vi "TimeConstantFilter_Example.vi"() -> ()   [LabVIEW 2019]
uses:
  <vilib>/Rock Robotics/WPI/ThirdParty/JAS_Junk/TrajLib/Trajectory_Library.lvlib
  <vilib>/Rock Robotics/WPI/ThirdParty/JAS_Junk/TrajLib/LinearFilter_LP_BW1_Execute.vi
  <vilib>/Rock Robotics/WPI/ThirdParty/JAS_Junk/TrajLib/LinearFilter_LP_BW2_Execute.vi
  <vilib>/Rock Robotics/WPI/ThirdParty/JAS_Junk/TrajLib/LinearFilter_HP_BW1_Execute.vi
  <vilib>/Rock Robotics/WPI/ThirdParty/JAS_Junk/TrajLib/LinearFilter_HP_BW2_Execute.vi
panel:
  out "Wait Adjust":dbl format="%11.3f"
  in  "Auto / Manual":bool=TRUE
  in  "Enable\nNoise":bool=TRUE
  in  "Filter Enable":bool=TRUE
  in  "Use White Noise":bool=TRUE
  in  "Tab Control 2":T1(tab)
  out "LP BW 2":cluster{dbl, dbl, "Output_Value":dbl}(graph)
  out "Butter 1 Out":dbl format="%11.3f"
  out "Low Pass Butterworth 1 Dial":dbl(knob)=-2.895988890827539e-05 scale=-20.0..20.0
  out "Curoff Freq\nLP BW 1":dbl format="%11.3f"
  out "LP BW 2":cluster{dbl, dbl, "Output_Value":dbl}(graph)
  out "Butter 2 Out":dbl format="%11.3f"
  out "Low Pass Butterworth 2 Dial":dbl(knob)=-2.895988890827539e-05 scale=-20.0..20.0
  out "Cutoff  Freq\nLP BW 2":dbl format="%11.3f"
  out "Curoff Freq\nHP BW 1":dbl format="%11.3f"
  out "HP BW 1":cluster{dbl, dbl, "Output_Value":dbl}(graph)
  out "HP BW 1":dbl format="%11.3f"
  out "High Pass Butterworth 1":dbl(knob)=-2.895988890827539e-05 scale=-20.0..20.0
  out "HP  BW 2":cluster{dbl, dbl, "Output_Value":dbl}(graph)
  out "Alt Lag":dbl format="%11.3f"
  out "High Pass Butterworth 2":dbl(knob)=-2.895988890827539e-05 scale=-20.0..20.0
  out "Cutoff Freq\nHP BW 2":dbl format="%11.3f"
  out "Duration":dbl format="%11.3f"
  out "Late":dbl format="%11.3f"
  in  "Manual\nInput":dbl(slide) min=-12.0 max=12.0 scale=-12.0..12.0
  out "Raw Noise":dbl(knob)=-2.895988890827539e-05 scale=-20.0..20.0
  out "Raw Noise":dbl format="%11.3f"
  out "Actual Input":dbl(knob)=-2.895988890827539e-05 scale=-20.0..20.0
  out "Actual Input":dbl format="%11.3f"
  in  "Time Const (Sec)":dbl=0.08 min=0.0 step=0.001 format="%10.4f"
  out "Input":cluster{"Manual\nInput":dbl, dbl, "f":dbl}(graph)
  out "Meas Dial":dbl(knob)=-2.895988890827539e-05 scale=-20.0..20.0
  out "Measured Value":dbl format="%11.3f"
  # "Linear (Time Constant) Filter Example"
  # "Loop Information"
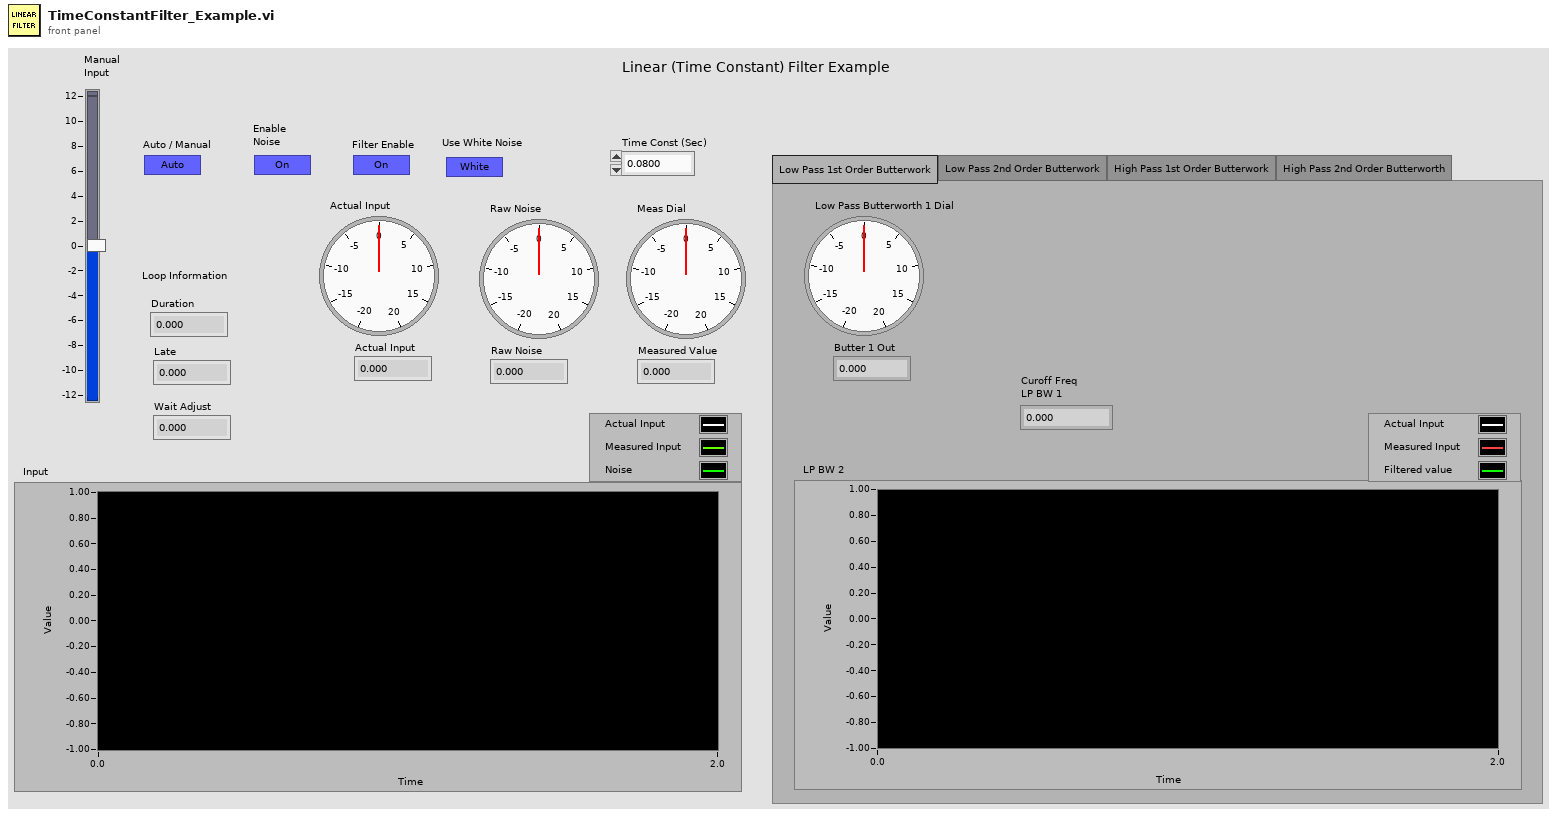
[diagram p1: front panel]
types:
  T1 = enum32{"Low Pass 1st Order Butterwork", "Low Pass 2nd Order Butterwork", "High Pass 1st Order Butterwork", "High Pass 2nd Order Butterworth"}
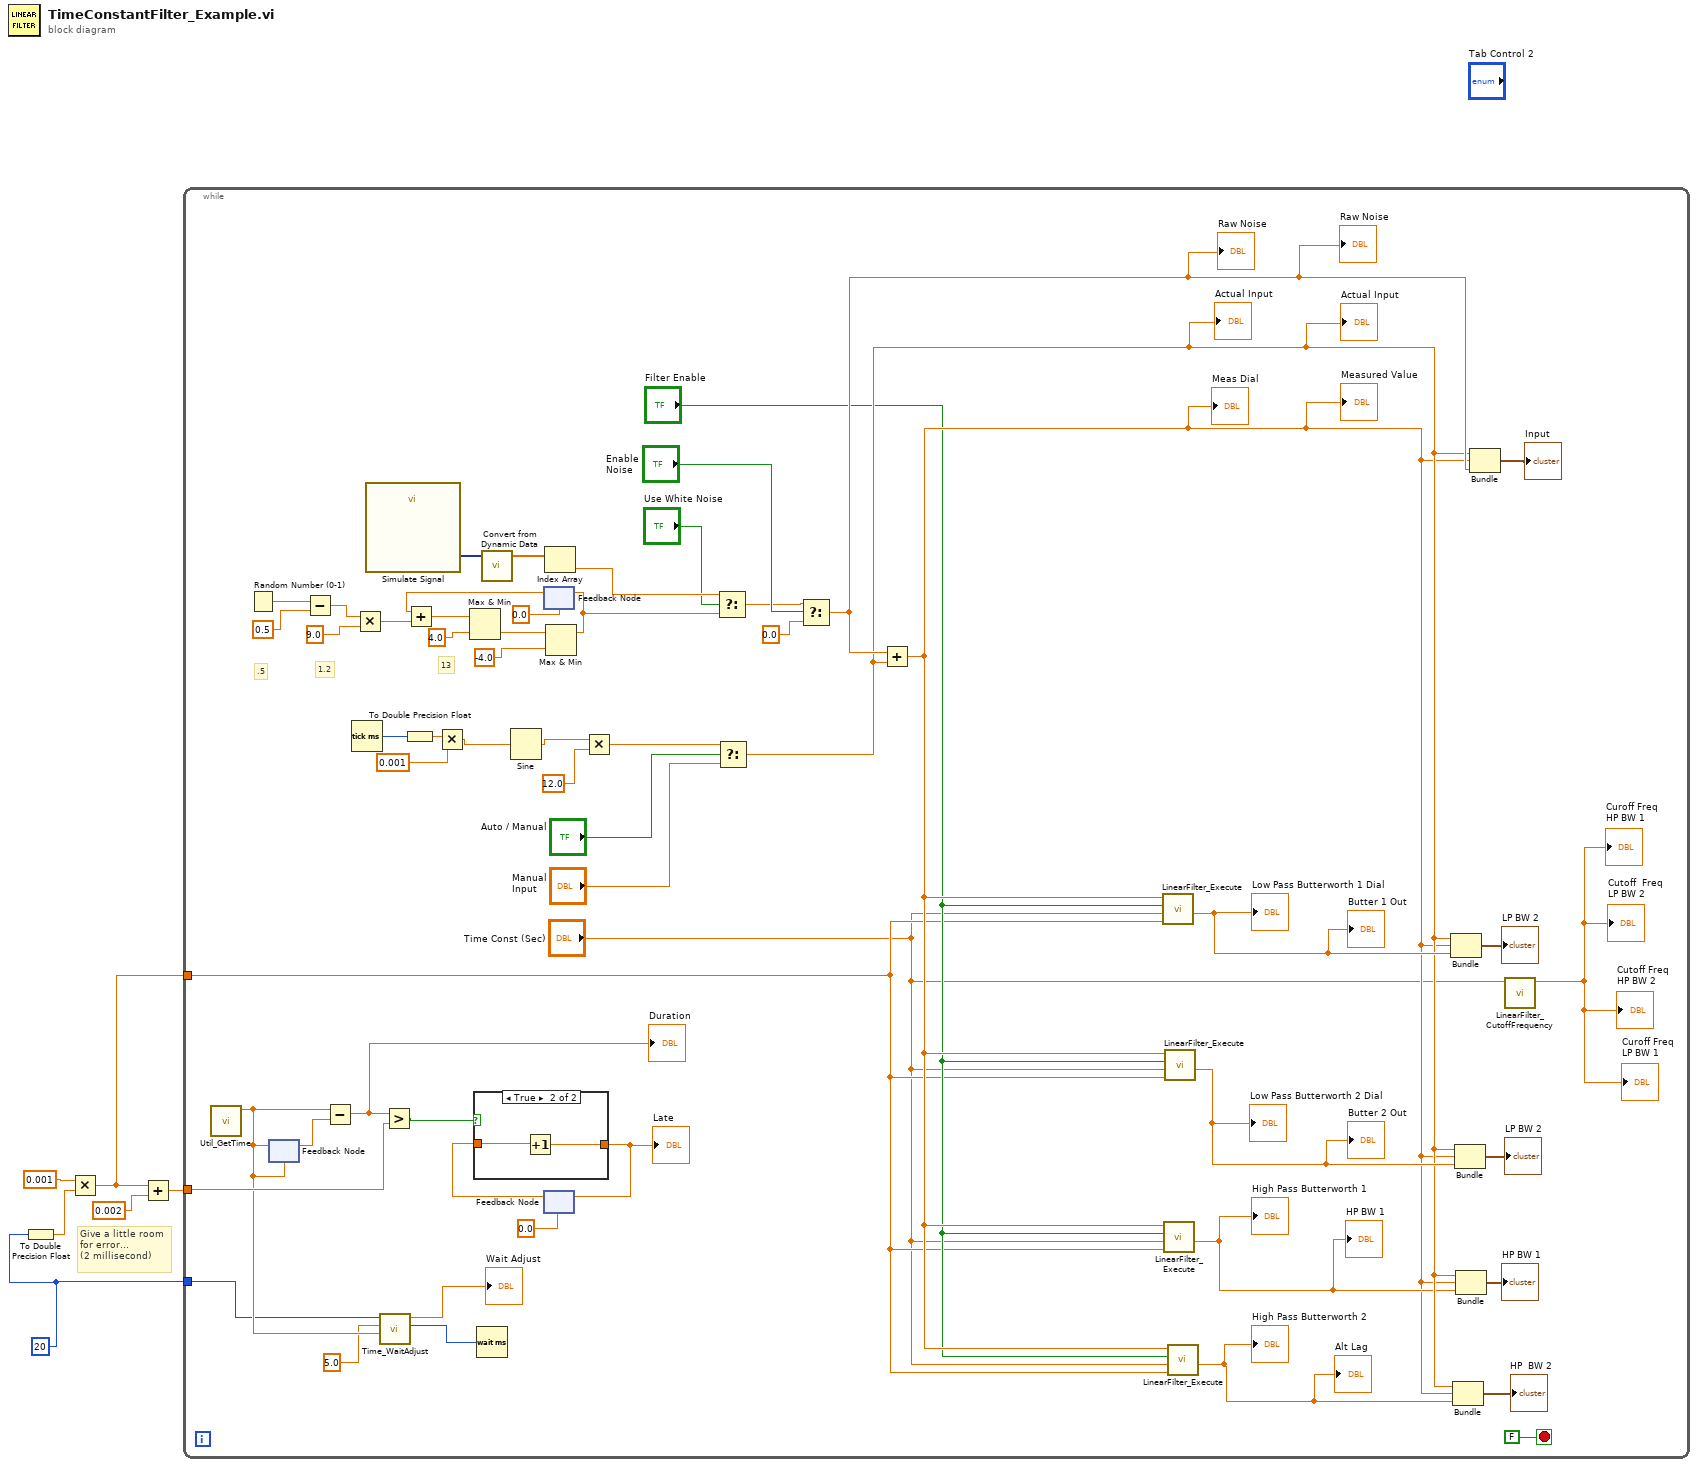
[diagram p0: block diagram]
diagram:
  w4 = u32 20 ("milliseconds to wait")
  # "Give a little room\nfor error...\n(2 millisecond)"
  n1 = To Double Precision Float(number=w4) -> (double precision float=w6:dbl)
  n2 = Multiply(x=0.001, y=w6) -> (x*y=w1:dbl)
  n3 = Add(x=w1, y=0.002) -> (x+y=w3:dbl)
  n4 = while {
    tunnel: w4 -> [w11]
    tunnel: w3 -> [w24]
    tunnel: w1 -> [w14]
    stop <- FALSE stop-if-true
    # "13"
    # "1.2"
    # ".5"
    n5 = call <vilib>:"Util_GetTime.vi"() -> ("FPGA_Time_Seconds"=w12:dbl)  [unwired: 9 in, 2 out]
    n6 = Random Number (0-1)() -> (number: 0 to 1=w58:dbl)
    n7 = feedback-in #1(w12) -> ()
    n8 = feedback #1(w12) -> (w27:dbl)
    n9 = Subtract(x=w58, y=0.5) -> (x-y=w54:dbl)
    n10 = Subtract(x=w12, y=w27) -> (x-y=w25:dbl)
    "Duration" <- w25
    n11 = Tick Count (ms)() -> (millisecond timer value=w51:u32)
    n12 = Multiply(x=w54, y=9.0) -> (x*y=w53:dbl)
    n13 = call "Simulate Signal"() -> ("DC with Uniform Noise"=w39:dynamicdata)  [unwired: 14 in, 1 out]
    n14 = call <vilib>:"Time_WaitAdjust.vi"("PassthroughTime_SEC"=w12, "MaxAdjustment_MS"=5.0 ("MaxDeviation_MS"), "DesiredLoopTime_MS"=w11) -> ("AdjustedWaitTime_MS"=w9:u32, "Offset_MS"=→"Wait Adjust":dbl)  [unwired: 7 in]
    n15 = Greater?(x=w25, y=w24) -> (0:w26:bool)
    n16 = To Double Precision Float(number=w51) -> (double precision float=w52:dbl)
    n17 = Multiply(x=w52, y=0.001) -> (x*y=w49:dbl)
    n18 = Wait (ms)(milliseconds to wait=w9) -> ()  [unwired: 1 out]
    n19 = call "Convert from Dynamic Data"("Dynamic Data Type"=w39) -> ("Array"=w38:dbl[])  [unwired: 3 in]
    n20 = Sine(x=w49) -> (sin(x)=w48:dbl)
    n21 = feedback #2(0.0) -> (w55:dbl)
    n22 = Add(x=w55, y=w53) -> (x+y=w57:dbl)
    n23 = Max & Min(x=w57, y=4.0) -> (min(x,y)=w56:dbl)  [unwired: 1 out]
    n24 = feedback #3(0.0) -> (w32:dbl)
    n25 = case shown="True" w26 {
      tunnel: [w64 w66] -> w33
      tunnel: w32 -> [w64 w65]
      frame False {
      }
      frame True {
        n26 = Increment(x=w65) -> (x+1=w66:dbl)
      }
    }
    "Late" <- w33
    n27 = feedback-in #3(w33) -> ()
    n28 = Index Array(array=w38) -> (element=w37:dbl)  [unwired: 1 in]
    n29 = Max & Min(x=w56, y=-4.0) -> (max(x,y)=w40:dbl)  [unwired: 1 out]
    n30 = feedback-in #2(w40) -> ()
    n31 = Multiply(x=w48, y=12.0) -> (x*y=w45:dbl)
    n32 = Select(t=w37, s="Use White Noise", f=w40) -> (s? t:f=w41:dbl)
    n33 = Select(t=w45, s="Auto / Manual", f="Manual\nInput") -> (s? t:f=w21:dbl)
    "Actual Input" <- w21
    "Actual Input" <- w21
    n34 = Select(t=w41, s="Enable\nNoise", f=0.0) -> (s? t:f=w35:dbl)
    "Raw Noise" <- w35
    "Raw Noise" <- w35
    n35 = Add(x=w35, y=w21) -> (x+y=w16:dbl)
    "Measured Value" <- w16
    "Meas Dial" <- w16
    n36 = call-poly <vilib>:"LinearFilter_Execute.vi"("SamplePeriod"=w14, "TimeConstant"="Time Const (Sec)", "Enable"="Filter Enable", "Input"=w16) -> ("Output"=w23:dbl)  [unwired: 7 in]
    "Butter 1 Out" <- w23
    "Low Pass Butterworth 1 Dial" <- w23
    n37 = call-poly <vilib>:"LinearFilter_Execute.vi"("SamplePeriod"=w14, "TimeConstant"="Time Const (Sec)", "Enable"="Filter Enable", "Input"=w16) -> ("Output"=w17:dbl)  [unwired: 7 in]
    "High Pass Butterworth 1" <- w17
    "HP BW 1" <- w17
    n38 = call-poly <vilib>:"LinearFilter_Execute.vi"("SamplePeriod"=w14, "TimeConstant"="Time Const (Sec)", "Enable"="Filter Enable", "Input"=w16) -> ("Output"=w22:dbl)  [unwired: 7 in]
    "Butter 2 Out" <- w22
    "Low Pass Butterworth 2 Dial" <- w22
    n39 = call-poly <vilib>:"LinearFilter_Execute.vi"("SamplePeriod"=w14, "TimeConstant"="Time Const (Sec)", "Enable"="Filter Enable", "Input"=w16) -> ("Output"=w18:dbl)  [unwired: 7 in]
    "Alt Lag" <- w18
    "High Pass Butterworth 2" <- w18
    n40 = Bundle("Manual\nInput"=w21, w16, "Output"=w23) -> (→"LP BW 2":cluster{"Manual\nInput":dbl, dbl, "Output":dbl})  [unwired: 1 in]
    n41 = Bundle("Manual\nInput"=w21, w16, "Output"=w18) -> (→"HP  BW 2":cluster{"Manual\nInput":dbl, dbl, "Output":dbl})  [unwired: 1 in]
    n42 = Bundle("Manual\nInput"=w21, w16, "Output"=w22) -> (→"LP BW 2":cluster{"Manual\nInput":dbl, dbl, "Output":dbl})  [unwired: 1 in]
    n43 = Bundle("Manual\nInput"=w21, w16, "Output"=w17) -> (→"HP BW 1":cluster{"Manual\nInput":dbl, dbl, "Output":dbl})  [unwired: 1 in]
    n44 = Bundle("Manual\nInput"=w21, w16, "f"=w35) -> (→"Input":cluster{"Manual\nInput":dbl, dbl, "f":dbl})  [unwired: 1 in]
    n45 = call <vilib>:"LinearFilter_CutoffFrequency.vi"("TimeConstant"="Time Const (Sec)") -> ("Cutoff Freq"=→"Cutoff Freq\nHP BW 2" →"Curoff Freq\nLP BW 1" →"Cutoff  Freq\nLP BW 2" →"Curoff Freq\nHP BW 1":dbl)  [unwired: 10 in]
  }
